vi "SetupCallBackEvents.vi"(8 "error in (no error)":errorcluster, 11 "DataGridView in":refnum<class "DataGridView.lvclass">) -> (0 "error out":errorcluster, 3 "DataGridView out":refnum<class "DataGridView.lvclass">)   [LabVIEW 2013, in "DataGrid.lvlib" / "DataGridView.lvclass"]
doc: "Callbacks are used to tie the .net grid events to the labview event structure and this VI sets the callback VIs up for each of the possible events for the grid class."
uses:
  DataGridView.lvclass
  System.Windows.Forms
  Events/Abstract EVENT/Abstract EVENT.lvclass
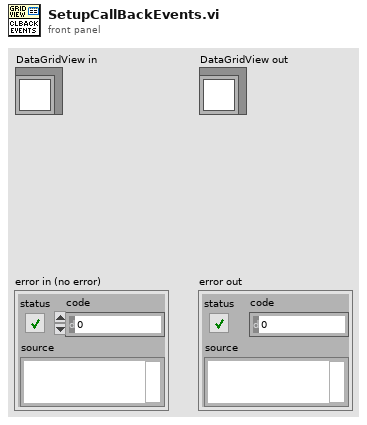
[diagram p1: front panel]
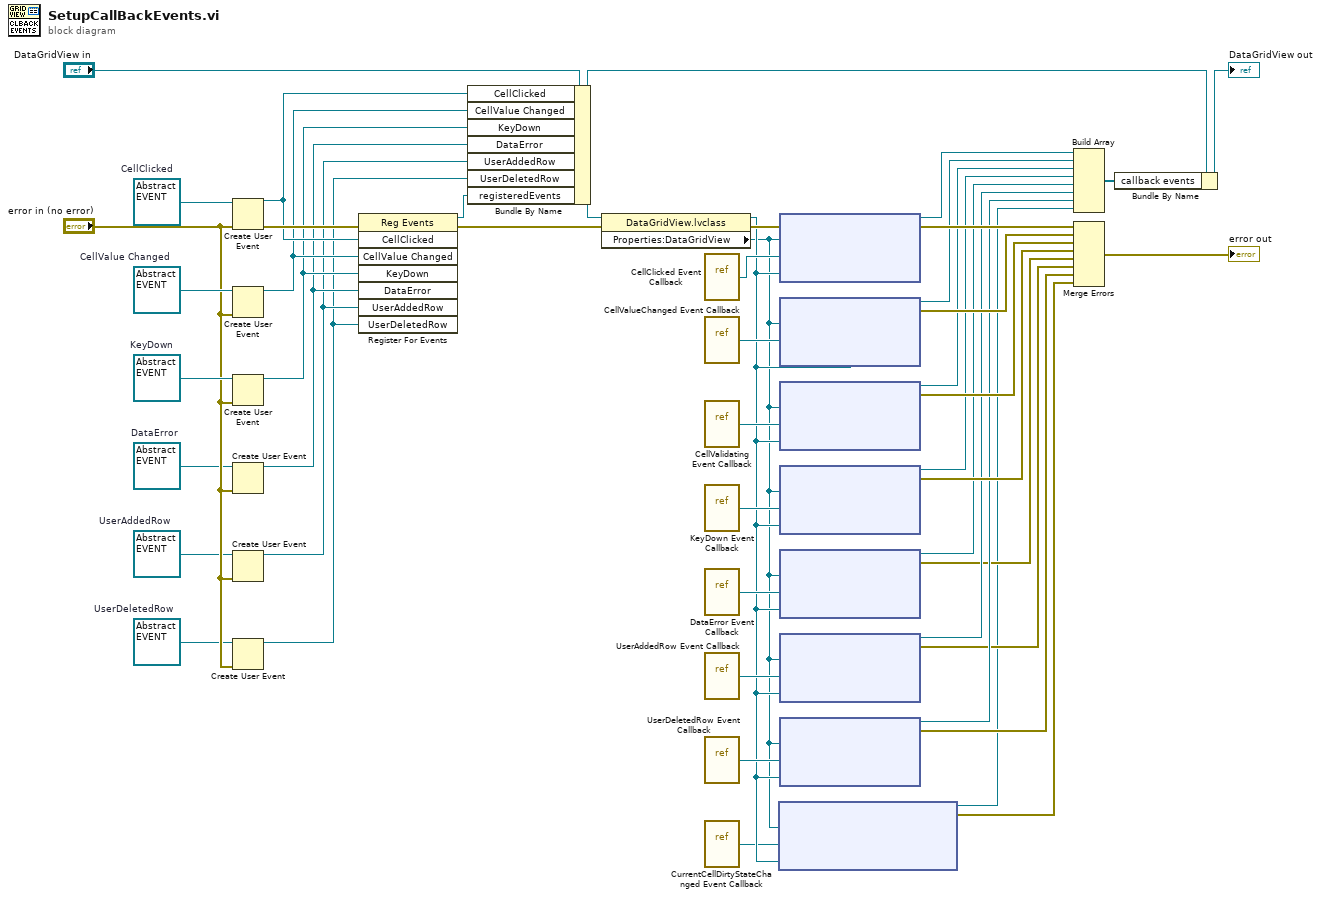
[diagram p0: block diagram]
diagram:
  w23 = refnum<class "Abstract EVENT.lvclass"> refnum  # UserDeletedRow
  w25 = refnum<class "Abstract EVENT.lvclass"> refnum  # UserAddedRow
  w24 = refnum<class "Abstract EVENT.lvclass"> refnum  # DataError
  w31 = refnum<class "Abstract EVENT.lvclass"> refnum  # KeyDown
  w35 = refnum<class "Abstract EVENT.lvclass"> refnum  # CellClicked
  w36 = refnum<class "Abstract EVENT.lvclass"> refnum  # CellValue Changed
  n1 = Create User Event(user event datatype=w35, error in="error in (no error)") -> (user event=w14:refnum<user-event>, error out=w48:errorcluster)
  n2 = Create User Event(user event datatype=w36, error in="error in (no error)") -> (user event=w13:refnum<user-event>)  [unwired: 1 out]
  n3 = Create User Event(user event datatype=w31, error in="error in (no error)") -> (user event=w12:refnum<user-event>)  [unwired: 1 out]
  n4 = Create User Event(user event datatype=w24, error in="error in (no error)") -> (user event=w11:refnum<user-event>)  [unwired: 1 out]
  n5 = Create User Event(user event datatype=w25, error in="error in (no error)") -> (user event=w10:refnum<user-event>)  [unwired: 1 out]
  n6 = Create User Event(user event datatype=w23, error in="error in (no error)") -> (user event=w9:refnum<user-event>)  [unwired: 1 out]
  n7 = register-events(error in=w48, w14, w13, w12, w11, w10, w9) -> (reference out=w7:refnum<event-registration>, error out=w46:errorcluster)  [unwired: 1 in]
  n8 = Bundle By Name(cluster="DataGridView in", "CellClicked"=w14, "CellValue Changed"=w13, "KeyDown"=w12, "DataError"=w11, "UserAddedRow"=w10, "UserDeletedRow"=w9, "registeredEvents"=w7) -> (w6:refnum<class "DataGridView.lvclass">)
  n9 = property class="DataGridView.lvclass"(reference=w6, error in=w46) -> (reference out=w5:refnum<class "DataGridView.lvclass">, error out=w47:errorcluster, "Properties:DataGridView"=w4:refnum<k24>)
  n10 = vi-ref "CellClicked Event Callback.vi"() -> ("vi reference"=w45:refnum<vi>)
  n11 = vi-ref "CellValueChanged Event Callback.vi"() -> ("vi reference"=w16:refnum<vi>)
  n12 = vi-ref "CellValidating Event Callback.vi"() -> ("vi reference"=w15:refnum<vi>)
  n13 = vi-ref "KeyDown Event Callback.vi"() -> ("vi reference"=w30:refnum<vi>)
  n14 = vi-ref "DataError Event Callback.vi"() -> ("vi reference"=w29:refnum<vi>)
  n15 = vi-ref "UserAddedRow Event Callback.vi"() -> ("vi reference"=w28:refnum<vi>)
  n16 = vi-ref "UserDeletedRow Event Callback.vi"() -> ("vi reference"=w27:refnum<vi>)
  n17 = vi-ref "CurrentCellDirtyStateChanged Event Callback.vi"() -> ("vi reference"=w3:refnum<vi>)
  n18 = node(w4, w3, w5) -> (w2:refnum<k27>, w1:errorcluster)  [unwired: 2 in]
  n19 = node(w47, w4, w45, w5) -> (w40:refnum<k27>, w44:errorcluster)  [unwired: 1 in]
  n20 = node(w4, w16, w5) -> (w41:refnum<k27>, w43:errorcluster)  [unwired: 2 in]
  n21 = node(w4, w15, w5) -> (w39:refnum<k27>, w34:errorcluster)  [unwired: 2 in]
  n22 = node(w4, w30, w5) -> (w32:refnum<k27>, w33:errorcluster)  [unwired: 2 in]
  n23 = node(w4, w29, w5) -> (w22:refnum<k27>, w19:errorcluster)  [unwired: 2 in]
  n24 = node(w4, w28, w5) -> (w21:refnum<k27>, w18:errorcluster)  [unwired: 2 in]
  n25 = node(w4, w27, w5) -> (w20:refnum<k27>, w17:errorcluster)  [unwired: 2 in]
  n26 = Build Array(w40, w41, w39, w32, w22, w21, w20, w2) -> (w37:refnum<k27>[])
  n27 = Merge Errors(w44, w43, w34, w33, w19, w18, w17, w1) -> (→"error out":errorcluster)
  n28 = Bundle By Name(cluster=w6, "callback events"=w37) -> (→"DataGridView out":refnum<class "DataGridView.lvclass">)
